vi "List Upgradable Packages.vi"(8 "error in":errorcluster, 10 "package name filter":string) -> (0 "error out":errorcluster, 2 "upgradable packages":string[][](table))   [LabVIEW 2014, in "NIPM_API.lvlib"]
doc: "Returns a list of upgradable packages and versions\n\nINPUT(s)\n<B>Package name filter</B>: Specifies the glob pattern (e.g. package-abc1, package-abc2, package-abc*, abc) used to filter the returned list of packages. If empty, this VI will return an unfiltered list of packages.\n\nOUTPUT(s)\n<B>Upgradable packages</B>: Outputs a 2D string array that lists the upgradable packages and the latest package versions to update to\nNote: This 2D array is unsorted.u"
uses:
  NIPM_API.lvlib
panel:
  out "cmd standard output":string
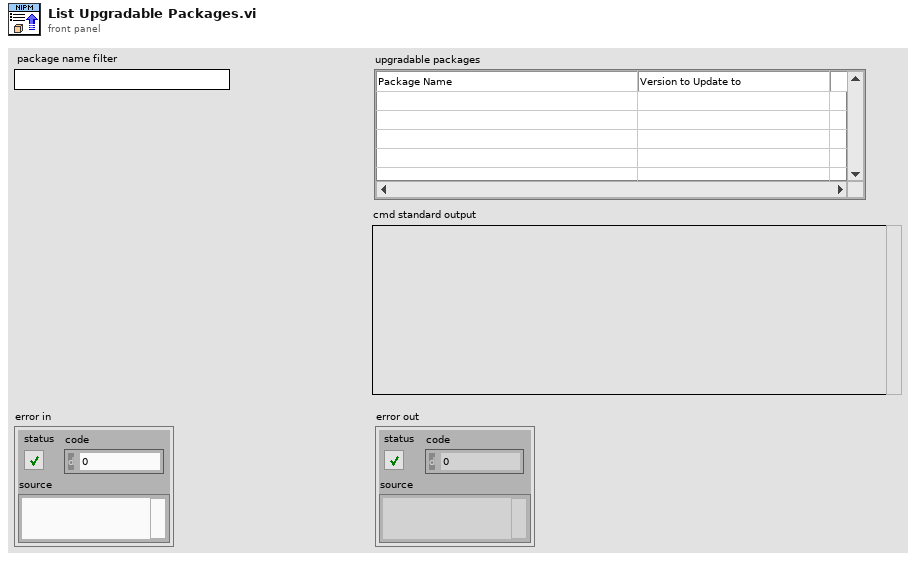
[diagram p1: front panel]
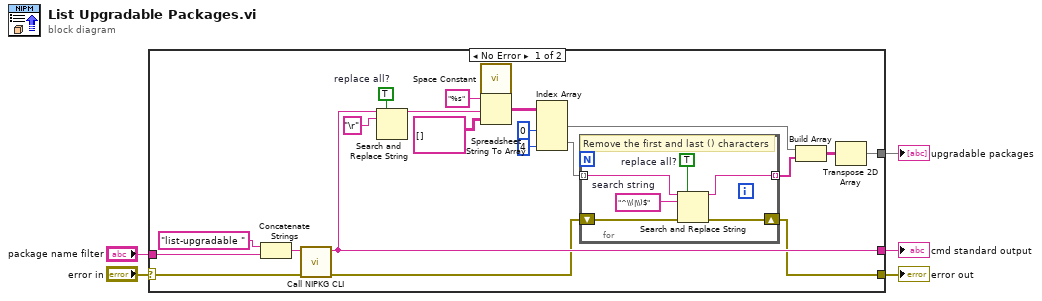
[diagram p0: block diagram]
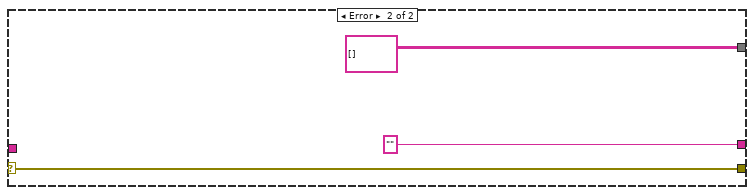
[diagram p2: hidden frame]
diagram:
  n1 = case shown="No Error" "error in" {
    selector: "error in" -> [w18 w35]
    tunnel: [w20 "" ("standard output")] -> w4
    tunnel: [w12 w35] -> w3
    tunnel: [w8 string[][] []] -> w2
    tunnel: "package name filter" -> [w6 _]
    frame No Error {
      w23 = TRUE  # replace all?
      n2 = Concatenate Strings("list-upgradable " ("format string"), w6) -> (w7:string)
      n3 = call "Call NIPKG CLI.vi"("error in (no error)"=w18, "command"=w7) -> ("error out"=w13:errorcluster, "command line standard output"=w20:string)  [unwired: 8 in]
      n4 = Search and Replace String(replace all?=w23, input string=w20, search string="\r") -> (result string=w25:string)  [unwired: 5 in, 3 out]
      n5 = call <vilib>:"Space Constant.vi"() -> ("String"=w17:string)
      n6 = Spreadsheet String To Array(delimiter (Tab)=w17, format string="%s", spreadsheet string=w25, array type (2D Dbl)=string[][] []) -> (array=w22:string[][])
      n7 = Index Array(array=w22, index (col) #1=0 ("disabled index (col)"), index (col) #2=4 ("index (col)")) -> (element #1=w10:string[], element #2=w14:string[])  [unwired: 2 in]
      n8 = for {
        tunnel: w14 -> [w32] mode=indexing
        shift-right: [w29] -> w12
        shift-left: w13 -> [w30]
        tunnel: [w28] -> w11 mode=indexing
        w27 = TRUE  # replace all?
        w31 = "^\\(|\\)$"  # search string
        # "Remove the first and last () characters"
        n9 = Search and Replace String(replace all?=w27, input string=w32, search string=w31, error in=w30) -> (result string=w28:string, error out=w29:errorcluster)  [unwired: 4 in, 2 out]
      }
      n10 = Build Array(w10, w11) -> (w9:string[][])
      n11 = Transpose 2D Array(2D array=w9) -> (transposed array=w8:string[][])
    }
    frame Error {
    }
  }
  "error out" <- w3
  "cmd standard output" <- w4
  "upgradable packages" <- w2
